vi "PlayQueue.vi"(0 "Program Interface in":refnum<class "Program Interface.lvclass">, 1 "robot":refnum<class "Universal Robot.lvclass">, 5 "error in (no error)":errorcluster, 9 "Subpanel":refnum<vi>) -> (14 "Program Interface out":refnum<class "Program Interface.lvclass">, 15 "programReturnStatus":T1=enum."Complete", 19 "error out":errorcluster)   [LabVIEW 2019, in "Program Interface.lvclass"]
uses:
  Program Interface.lvclass
  Robot/Universal Robot/Universal Robot.lvclass
  Robot/Universal Robot/ProgramReturnStatus.ctl
  Program Interface.lvclass/Program Interface.ctl
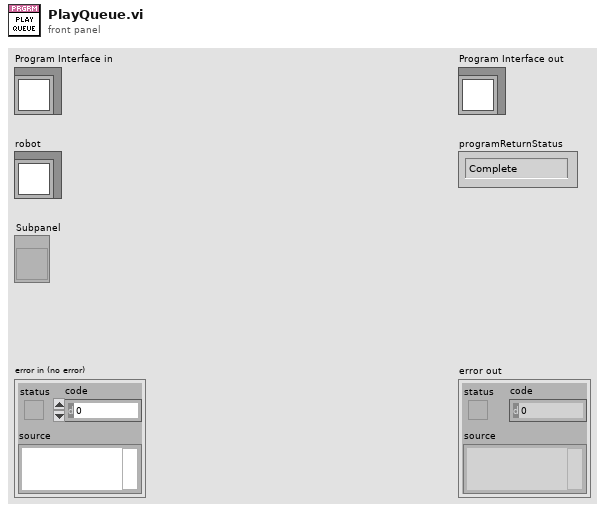
[diagram p1: front panel]
types:
  T1 = typedef "Universal Robot.lvclass/ProgramReturnStatus.ctl" = enum16{"Incomplete", "Complete", "Stopped", "User Stopped", "Error", "Faulted", "Timeout"}
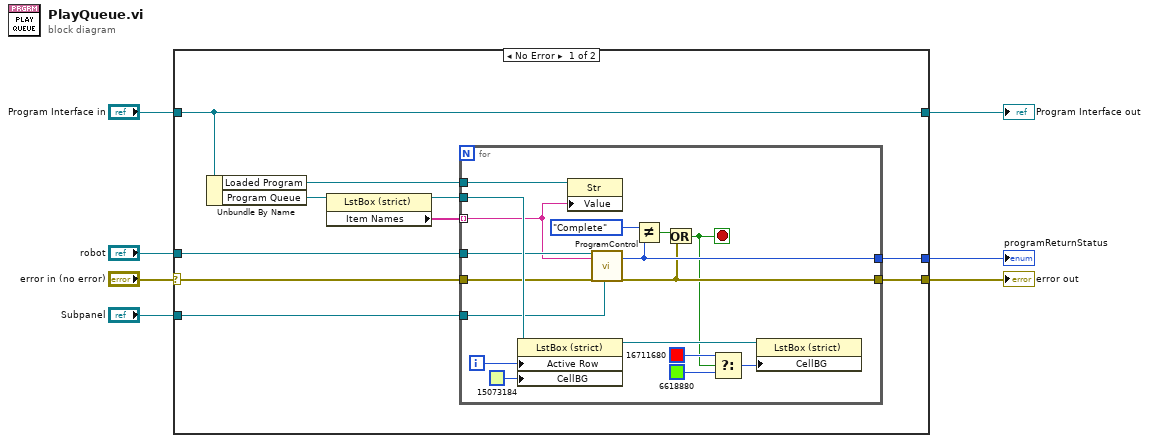
[diagram p0: block diagram]
diagram:
  n1 = case shown="No Error" "error in (no error)" {
    selector: "error in (no error)" -> [w16 w36]
    tunnel: [w15 w36] -> w6
    tunnel: [w17 w35] -> w4
    tunnel: "Program Interface in" -> [w17 w35]
    tunnel: "robot" -> [w12 _]
    tunnel: [w9 _] -> w2
    tunnel: "Subpanel" -> [w8 _]
    frame No Error {
      n2 = Unbundle By Name(w17) -> ("Loaded Program"=w11:refnum<vi>, "Program Queue"=w14:refnum<vi>)
      n3 = property class="LstBox (strict)"(reference=w14) -> (reference out=w10:refnum<vi>, "Item Names"=w13:string[])  [unwired: 1 in, 1 out]
      n4 = for {
        tunnel: w13 -> [w25] mode=indexing
        tunnel: w12 -> [w26]
        tunnel: w16 -> [w24]
        tunnel: [w19] -> w15
        tunnel: w11 -> [w34]
        tunnel: w10 -> [w33]
        tunnel: [w22] -> w9
        tunnel: w8 -> [w23]
        i -> [w32]
        stop <- w18 stop-if-true
        n5 = property class="LstBox (strict)"(reference=w33, "Active Row"=w32, "CellBG"=u32 15073184) -> (reference out=w30:refnum<vi>)  [unwired: 1 in, 1 out]
        n6 = property class="Str"(reference=w34, "Value"=w25) -> ()  [unwired: 1 in, 2 out]
        n7 = call-dynamic "ProgramControl.vi"("Universal Robot.lvclass in"=w26, "Program"=w25, "error in (no error)"=w24, "Subpanel"=w23) -> ("programReturnStatus"=w22:T1, "error out"=w19:errorcluster)  [unwired: 13 in, 1 out]
        n8 = Not Equal?(x=ProgramReturnStatus."Complete", y=w22) -> (x != y?=w20:bool)
        n9 = Or(x=w20, y=w19) -> (x .or. y?=w18:bool)
        n10 = Select(t=u32 16711680, s=w18, f=u32 6618880) -> (s? t:f=w27:u32)
        n11 = property class="LstBox (strict)"(reference=w30, "CellBG"=w27) -> ()  [unwired: 1 in, 2 out]
      }
    }
    frame Error {
    }
  }
  "error out" <- w6
  "Program Interface out" <- w4
  "programReturnStatus" <- w2
